vi "Create.vi"   [LabVIEW 2018, in "Toolkit.lvlib" / "File Info.lvclass"]
doc: "Creates a new File Info object that represents a libssh2lv shared library File Info struct. This VI must be called, or executed, before using any other File Info-related VIs. This VI allocates memory within the libssh2lv shared library that must be explicitly deallocated, or freed, at the end of the application using the <B>Destroy</B> VI to avoid memory leaks or running Out-of-Memory (OOM) on a resource contrained system.\n\nA File Info object represents the read-only information obtained about a remote SSH server file."
uses:
  File Info.lvclass
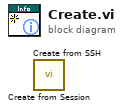
[diagram p0: block diagram]
diagram:
  n1 = call "Create from Session.vi"() -> ()  [unwired: 9 in, 3 out]
  n2 = call "Create from SSH.vi"() -> ()  [unwired: 10 in, 2 out]
